vi "get_value_for_inline_table.vi"(8 "error in (no error)":errorcluster, 11 "Value in":refnum<class "Value.lvclass">) -> (0 "error out":errorcluster, 3 "InlineTable out":refnum<class "InlineTable.lvclass">)   [LabVIEW 2020, in "toml_edit.lvlib" / "Value.lvclass"]
uses:
  Value.lvclass
  InlineTable/InlineTable.lvclass
  value_type--enum.ctl
  Value.lvclass/Value.ctl
  dragon_toml_64.dll
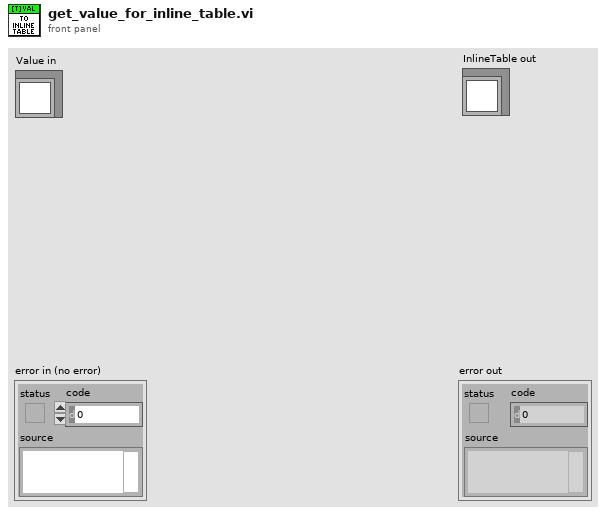
[diagram p1: front panel]
types:
  T1 = typedef "toml_edit.lvlib/Value.lvclass/value_type--enum.ctl" = enum16{"Unknown", "String", "Integer", "Float", "Boolean", "Datetime", "Array", "InlineTable"}
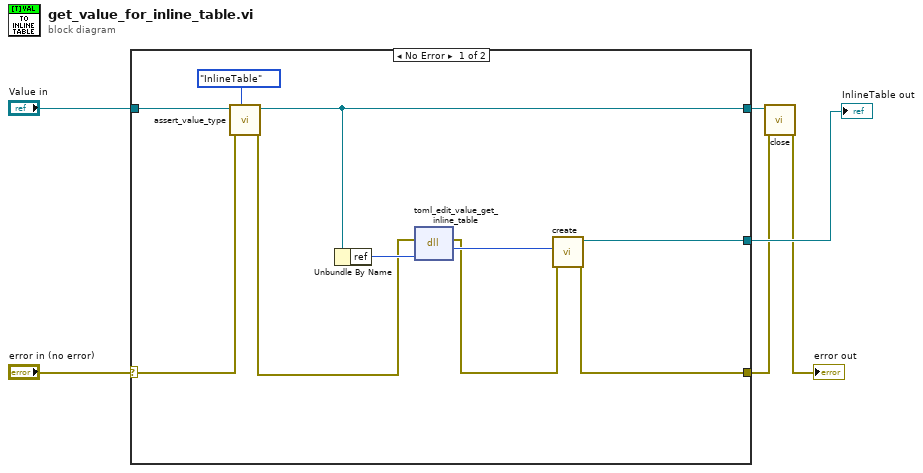
[diagram p0: block diagram]
diagram:
  n1 = case shown="No Error" "error in (no error)" {
    selector: "error in (no error)" -> [w9 w18]
    tunnel: [w13 w18] -> w2
    tunnel: [w11 w17] -> w3
    tunnel: "Value in" -> [w10 w17]
    tunnel: [w14 _] -> w4
    frame No Error {
      n2 = call "assert_value_type.vi"("value_type"=value_type--enum."InlineTable", "error in (no error)"=w9, "Value in"=w10) -> ("error out"=w8:errorcluster, "Value out"=w11:refnum<class "Value.lvclass">)  [unwired: 7 in]
      n3 = Unbundle By Name(w11) -> ("ref"=w16:u64)
      n4 = dll-call lib="C:/projects/dragon-desktop/source/submodules/toml-edit-labview/lv_src/dragon_toml_*.*" fn="toml_edit_value_get_inline_table"(error in=w8, "item_ref"=w16) -> (error out=w12:errorcluster, "table_ptr"=w15:u64)  [unwired: 3 in, 1 out]
      n5 = call "create.vi"("error in (no error)"=w12, "ref"=w15) -> ("error out"=w13:errorcluster, "InlineTable out"=w14:refnum<class "InlineTable.lvclass">)  [unwired: 8 in]
    }
    frame Error {
    }
  }
  "InlineTable out" <- w4
  n6 = call "close.vi"("error in (no error)"=w2, "Value in"=w3) -> ("error out"=→"error out":errorcluster)  [unwired: 9 in]
